vi "Tool Objects.vi"(8 "error in (no error)":errorcluster, 11 "Tool Data in":refnum<class "Tool Data.lvclass">) -> (0 "error out":errorcluster, 3 "Tool Data out":refnum<class "Tool Data.lvclass">)   [LabVIEW 2019, in "Tool Data.lvclass"]
uses:
  Tool Data.lvclass
  Tool Data.lvclass/Tool Data.ctl
  Tool Dot/Tool Dots.lvclass
  Tool Rectangle/Tool Rectangle.lvclass
  Tool Path/Tool Path.lvclass
  Tool Funnel/Tool Funnel.lvclass
panel:
  out "XY Graph":cluster{"X":dbl, "Y":dbl}[](graph)
  out "Dots":u32
  out "Rect":u32
  out "Funnel":u32
  out "Path":u32
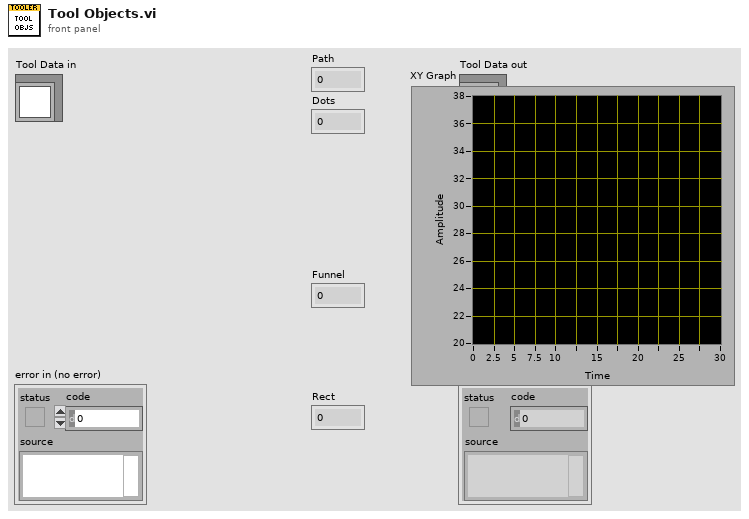
[diagram p1: front panel]
types:
  T1 = cluster{"Changed":bool, "index of element":i32}[]
  T2 = typedef "Setting Database.lvclass/PublicEvents--Setting Database.RectanglesUpdated.ctl" = refnum<class "Rectangle Settings.lvclass">[]
  T3 = typedef "Setting Database.lvclass/PublicEvents--Setting Database.FunnelsUpdated.ctl" = refnum<class "Funnel Settings.lvclass">[]
  T4 = typedef "Setting Database.lvclass/PublicEvents--Setting Database.PathsUpdated.ctl" = refnum<class "Path Settings.lvclass">[]
  T5 = typedef "Setting Database.lvclass/PublicEvents--Setting Database.DotsUpdated.ctl" = refnum<class "Dot Settings.lvclass">[]
  T6 = typedef "Points.ctl" = cluster{"X":dbl, "Y":dbl}[]
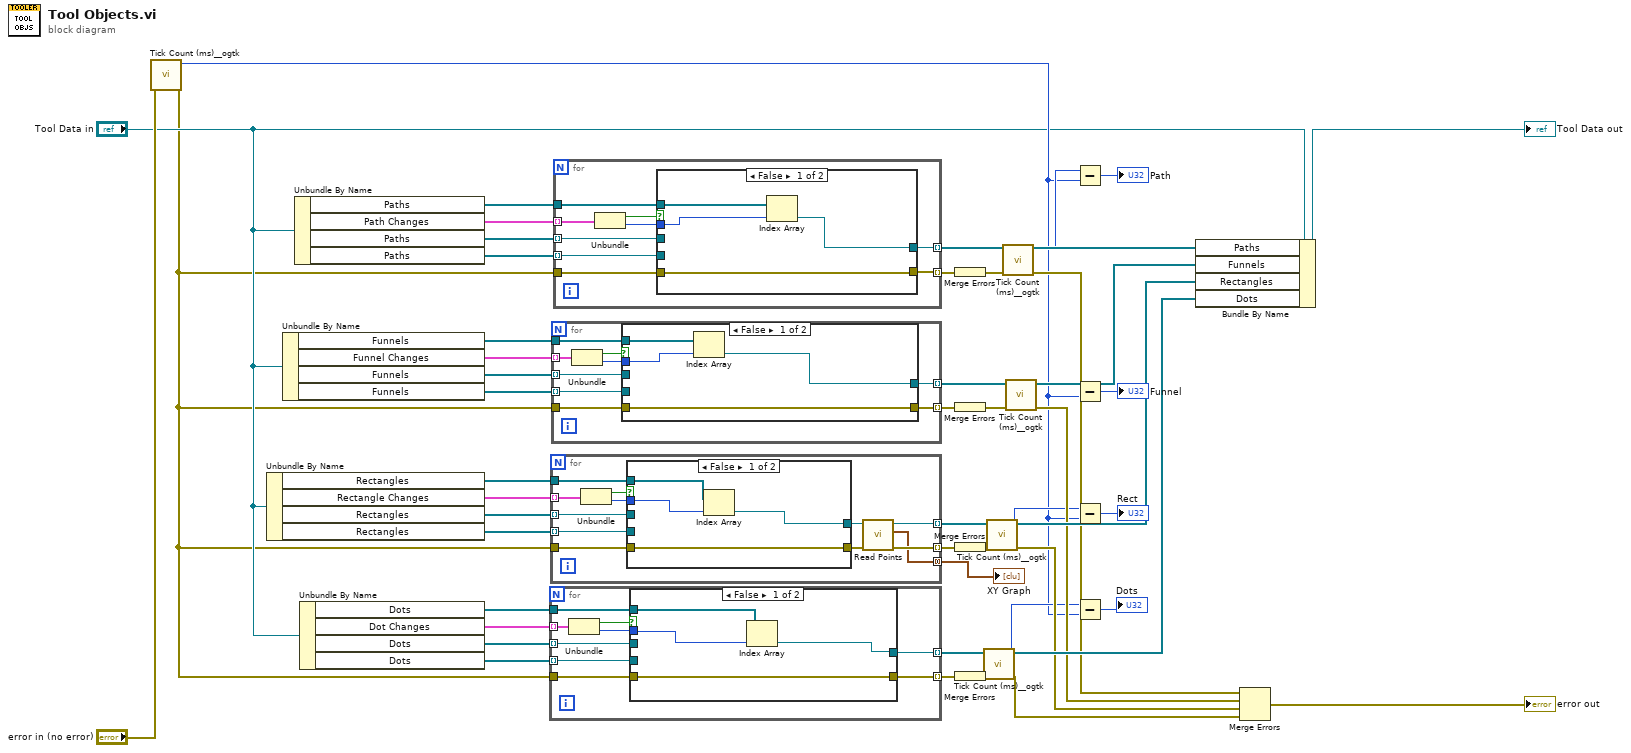
[diagram p0: block diagram]
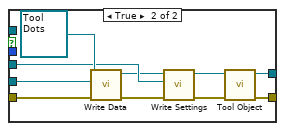
[diagram p2: hidden frame]
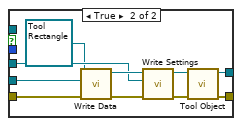
[diagram p3: hidden frame]
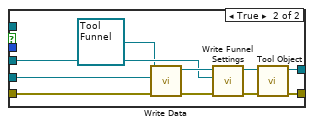
[diagram p4: hidden frame]
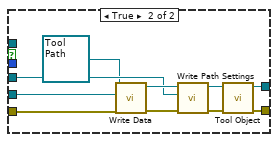
[diagram p5: hidden frame]
diagram:
  n1 = call <userlib>:"Tick Count (ms)__ogtk.vi"("error in (no error)"="error in (no error)") -> ("error out"=w1:errorcluster, "millisecond timer value"=w14:u32)  [unwired: 9 in]
  n2 = Unbundle By Name("Tool Data in") -> ("Rectangles"=w6:refnum<class "Tool Rectangle.lvclass">[], "Rectangle Changes"=w5:T1, "Rectangles"=w43:T2, "Rectangles"=w42:refnum<class "Rectangle.lvclass">[])
  n3 = Unbundle By Name("Tool Data in") -> ("Funnels"=w7:refnum<class "Tool Funnel.lvclass">[], "Funnel Changes"=w8:T1, "Funnels"=w44:T3, "Funnels"=w45:refnum<class "Path.lvclass">[])
  n4 = Unbundle By Name("Tool Data in") -> ("Paths"=w10:refnum<class "Tool Path.lvclass">[], "Path Changes"=w9:T1, "Paths"=w47:T4, "Paths"=w46:refnum<class "Path.lvclass">[])
  n5 = Unbundle By Name("Tool Data in") -> ("Dots"=w4:refnum<class "Tool Dots.lvclass">[], "Dot Changes"=w3:T1, "Dots"=w36:T5, "Dots"=w35:refnum<class "Dot.lvclass">[])
  n6 = for {
    tunnel: w36 -> [w55] mode=indexing
    tunnel: w35 -> [w56] mode=indexing
    tunnel: w1 -> [w54]
    tunnel: [w53] -> w27 mode=indexing
    tunnel: [w52] -> w34 mode=indexing
    tunnel: w4 -> [w48]
    tunnel: w3 -> [w51] mode=indexing
    n7 = Unbundle(w51) -> ("Changed"=w50:bool, "index of element"=w49:i32)
    n8 = case shown="False" w50 {
      tunnel: w56 -> [_ w69]
      tunnel: w55 -> [_ w68]
      tunnel: w54 -> [w57 w66]
      tunnel: [w57 w63] -> w53
      tunnel: [w58 w61] -> w52
      tunnel: w49 -> [w59 _]
      tunnel: w48 -> [w60 _]
      frame False {
        n9 = Index Array(array=w60, index=w59) -> (element=w58:refnum<class "Tool Dots.lvclass">)
      }
      frame True {
        n10 = call-dynamic "Write Data.vi"("error in (no error)"=w66, "Dot.lvclass"=w69, "Tool Dots in"=refnum<class "Tool Dots.lvclass"> refnum) -> ("error out"=w65:errorcluster, "Tool Dots out"=w67:refnum<class "Tool Dots.lvclass">)  [unwired: 7 in]
        n11 = call-dynamic "Write Settings.vi"("error in (no error)"=w65, "Dot Settings.lvclass"=w68, "Tool Dots in"=w67) -> ("error out"=w64:errorcluster, "Tool Dots out"=w62:refnum<class "Tool Dots.lvclass">)  [unwired: 7 in]
        n12 = call-dynamic "Tool Object.vi"("error in (no error)"=w64, "Tool Dots in"=w62) -> ("error out"=w63:errorcluster, "Tool Dots out"=w61:refnum<class "Tool Dots.lvclass">)  [unwired: 8 in]
      }
    }
  }
  n13 = for {
    tunnel: w43 -> [w79] mode=indexing
    tunnel: w42 -> [w80] mode=indexing
    tunnel: [w76] -> w38 mode=indexing
    tunnel: w1 -> [w78]
    tunnel: [w81] -> w29 mode=indexing
    tunnel: [w75] -> w11 mode=concatenating
    tunnel: w6 -> [w71]
    tunnel: w5 -> [w74] mode=indexing
    n14 = Unbundle(w74) -> ("Changed"=w73:bool, "index of element"=w72:i32)
    n15 = case shown="False" w73 {
      tunnel: [w82 w95] -> w81
      tunnel: w80 -> [_ w90]
      tunnel: w79 -> [_ w89]
      tunnel: w78 -> [w82 w88]
      tunnel: [w83 w86] -> w77
      tunnel: w72 -> [w84 _]
      tunnel: w71 -> [w85 _]
      frame False {
        n16 = Index Array(array=w85, index=w84) -> (element=w83:refnum<class "Tool Rectangle.lvclass">)
      }
      frame True {
        n17 = call-dynamic "Write Data.vi"("error in (no error)"=w88, "Rectangle.lvclass"=w90, "Tool Rectangle in"=refnum<class "Tool Rectangle.lvclass"> refnum) -> ("error out"=w93:errorcluster, "Tool Rectangle out"=w94:refnum<class "Tool Rectangle.lvclass">)  [unwired: 7 in]
        n18 = call-dynamic "Write Settings.vi"("error in (no error)"=w93, "Rectangle Settings.lvclass"=w89, "Tool Rectangle in"=w94) -> ("error out"=w91:errorcluster, "Tool Rectangle out"=w92:refnum<class "Tool Rectangle.lvclass">)  [unwired: 7 in]
        n19 = call-dynamic "Tool Object.vi"("error in (no error)"=w91, "Tool Rectangle in"=w92) -> ("error out"=w95:errorcluster, "Tool Rectangle out"=w86:refnum<class "Tool Rectangle.lvclass">)  [unwired: 8 in]
      }
    }
    n20 = call-dynamic "Read Points.vi"("Tool Object in"=w77) -> ("Points"=w75:T6, "Tool Object out"=w76:refnum<class "Tool Rectangle.lvclass">)  [unwired: 8 in, 1 out]
  }
  "XY Graph" <- w11
  n21 = for {
    tunnel: w44 -> [w102] mode=indexing
    tunnel: w45 -> [w103] mode=indexing
    tunnel: [w100] -> w39 mode=indexing
    tunnel: w1 -> [w104]
    tunnel: [w101] -> w31 mode=indexing
    tunnel: w8 -> [w99] mode=indexing
    tunnel: w7 -> [w96]
    n22 = Unbundle(w99) -> ("Changed"=w98:bool, "index of element"=w97:i32)
    n23 = case shown="False" w98 {
      tunnel: w104 -> [w105 w115]
      tunnel: w103 -> [_ w113]
      tunnel: w102 -> [_ w112]
      tunnel: [w105 w111] -> w101
      tunnel: [w106 w110] -> w100
      tunnel: w97 -> [w107 _]
      tunnel: w96 -> [w108 _]
      frame False {
        n24 = Index Array(array=w108, index=w107) -> (element=w106:refnum<class "Tool Funnel.lvclass">)
      }
      frame True {
        n25 = call-dynamic "Write Data.vi"("error in (no error)"=w115, "Path.lvclass"=w113, "Tool Path in"=refnum<class "Tool Funnel.lvclass"> refnum ("Tool Funnel in")) -> ("error out"=w118:errorcluster, "Tool Path out"=w114:refnum<class "Tool Funnel.lvclass">)  [unwired: 7 in]
        n26 = call-dynamic "Write Funnel Settings.vi"("error in (no error)"=w118, "Funnel Settings.lvclass"=w112, "Tool Funnel in"=w114) -> ("error out"=w116:errorcluster, "Tool Funnel out"=w117:refnum<class "Tool Funnel.lvclass">)  [unwired: 7 in]
        n27 = call-dynamic "Tool Object.vi"("error in (no error)"=w116, "Tool Funnel in"=w117) -> ("error out"=w111:errorcluster, "Tool Funnel out"=w110:refnum<class "Tool Funnel.lvclass">)  [unwired: 8 in]
      }
    }
  }
  n28 = for {
    tunnel: w47 -> [w125] mode=indexing
    tunnel: w46 -> [w126] mode=indexing
    tunnel: [w123] -> w40 mode=indexing
    tunnel: w1 -> [w127]
    tunnel: [w124] -> w33 mode=indexing
    tunnel: w10 -> [w122]
    tunnel: w9 -> [w121] mode=indexing
    n29 = Unbundle(w121) -> ("Changed"=w120:bool, "index of element"=w119:i32)
    n30 = case shown="False" w120 {
      tunnel: w127 -> [w128 w138]
      tunnel: w126 -> [_ w137]
      tunnel: w125 -> [_ w136]
      tunnel: [w128 w134] -> w124
      tunnel: [w129 w133] -> w123
      tunnel: w122 -> [w131 _]
      tunnel: w119 -> [w130 _]
      frame False {
        n31 = Index Array(array=w131, index=w130) -> (element=w129:refnum<class "Tool Path.lvclass">)
      }
      frame True {
        n32 = call-dynamic "Write Data.vi"("error in (no error)"=w138, "Path.lvclass"=w137, "Tool Path in"=refnum<class "Tool Path.lvclass"> refnum) -> ("error out"=w140:errorcluster, "Tool Path out"=w141:refnum<class "Tool Path.lvclass">)  [unwired: 7 in]
        n33 = call-dynamic "Write Path Settings.vi"("error in (no error)"=w140, "Path Settings.lvclass"=w136, "Tool Path in"=w141) -> ("error out"=w135:errorcluster, "Tool Path out"=w139:refnum<class "Tool Path.lvclass">)  [unwired: 7 in]
        n34 = call-dynamic "Tool Object.vi"("error in (no error)"=w135, "Tool Path in"=w139) -> ("error out"=w134:errorcluster, "Tool Path out"=w133:refnum<class "Tool Path.lvclass">)  [unwired: 8 in]
      }
    }
  }
  n35 = Merge Errors(w33) -> (w32:errorcluster)
  n36 = Merge Errors(w31) -> (w30:errorcluster)
  n37 = Merge Errors(w29) -> (w28:errorcluster)
  n38 = Merge Errors(w27) -> (w26:errorcluster)
  n39 = call <userlib>:"Tick Count (ms)__ogtk.vi"("error in (no error)"=w26) -> ("error out"=w22:errorcluster, "millisecond timer value"=w15:u32)  [unwired: 9 in]
  n40 = call <userlib>:"Tick Count (ms)__ogtk.vi"("error in (no error)"=w28) -> ("error out"=w23:errorcluster, "millisecond timer value"=w16:u32)  [unwired: 9 in]
  n41 = call <userlib>:"Tick Count (ms)__ogtk.vi"("error in (no error)"=w32) -> ("error out"=w25:errorcluster, "millisecond timer value"=w18:u32)  [unwired: 9 in]
  n42 = call <userlib>:"Tick Count (ms)__ogtk.vi"("error in (no error)"=w30) -> ("error out"=w24:errorcluster, "millisecond timer value"=w17:u32)  [unwired: 9 in]
  n43 = Subtract(x=w18, y=w14) -> (x-y=→"Path":u32)
  n44 = Subtract(x=w17, y=w14) -> (x-y=→"Funnel":u32)
  n45 = Subtract(x=w16, y=w14) -> (x-y=→"Rect":u32)
  n46 = Subtract(x=w15, y=w14) -> (x-y=→"Dots":u32)
  n47 = Bundle By Name(cluster="Tool Data in", "Paths"=w40, "Funnels"=w39, "Rectangles"=w38, "Dots"=w34) -> (→"Tool Data out":refnum<class "Tool Data.lvclass">)
  n48 = Merge Errors(w25, w24, w23, w22) -> (→"error out":errorcluster)
